vi "2636 EPSC LTP LTD Cycles.vi"() -> ()   [LabVIEW 2023]
uses:
  <instrlib>/Keithley 2600 Series/Public/Channel.ctl
  <instrlib>/Keithley 2600 Series/Keithley 2600 Series.lvlib
  <userlib>/_OpenG.lib/time/time.llb/openg_time.lvlib
panel:
  in  "Cycle Number":u32=50
  in  "LTD Pulse Level (V)":dbl=-10.0
  in  "error in (no error)":errorcluster
  in  "Log Time After Pulses (s)":dbl=0.5 format="%#_13g"
  in  "Log Time Before Pulses (s)":dbl=0.5 format="%#_13g"
  in  "Auto Enable Output":bool=TRUE
  in  "Reset":bool=TRUE
  in  "Error Query":bool
  out "Pulsed IV Filename Out":path caption="Filename Out"
  in  "Pulsed IV Filename":path=path "C:/Data/pulse_I_V.lvm" caption="Filename"
  out "Pulse IV":cluster{"X":dbl[], "Y":dbl[]}[](graph)
  out "I_ds Log Filename Out":path caption="Filename Out"
  in  "I_ds Log Filename":path=path "C:/Data/I_ds_vs_time.lvm" caption="Filename"
  out "Data":dbl[](array[numeric])
  out "Result Chart":dynamicdata(graph)
  out "error out":errorcluster
  out "Complete?":bool
  out "Overflow?":bool
  in  "Stop":bool
  in  "Pulse Duration (s)":dbl=0.01
  in  "Post-Pulse Duration (s)":dbl=0.05
  in  "Pre-Pulse Duration (s)":dbl=0.05
  in  "Buffer size":u32=1024
  in  "LT Pulse Number":u32=50
  in  "Drain Source Channel":T1=enum."Channel B"
  in  "V_ds(V)":dbl=0.01
  in  "I_ds NPLC":dbl=0.1
  in  "I_ds Range (A)":dbl=1e-06
  in  "I pulse Range (A)":dbl=1e-06
  in  "I pulse NPLC":dbl=0.1
  in  "LTP Pulse Level (V)":dbl=10.0
  in  "Pulse Channel":T1
  in  "2636 Address":refnum<visa-resource-name>="GPIB0::26::INSTR"
  # "Synaptic EPSC LTP-LTD Cycle Test (Three-terminal Devices)"
  # "by JHC (20250322)"
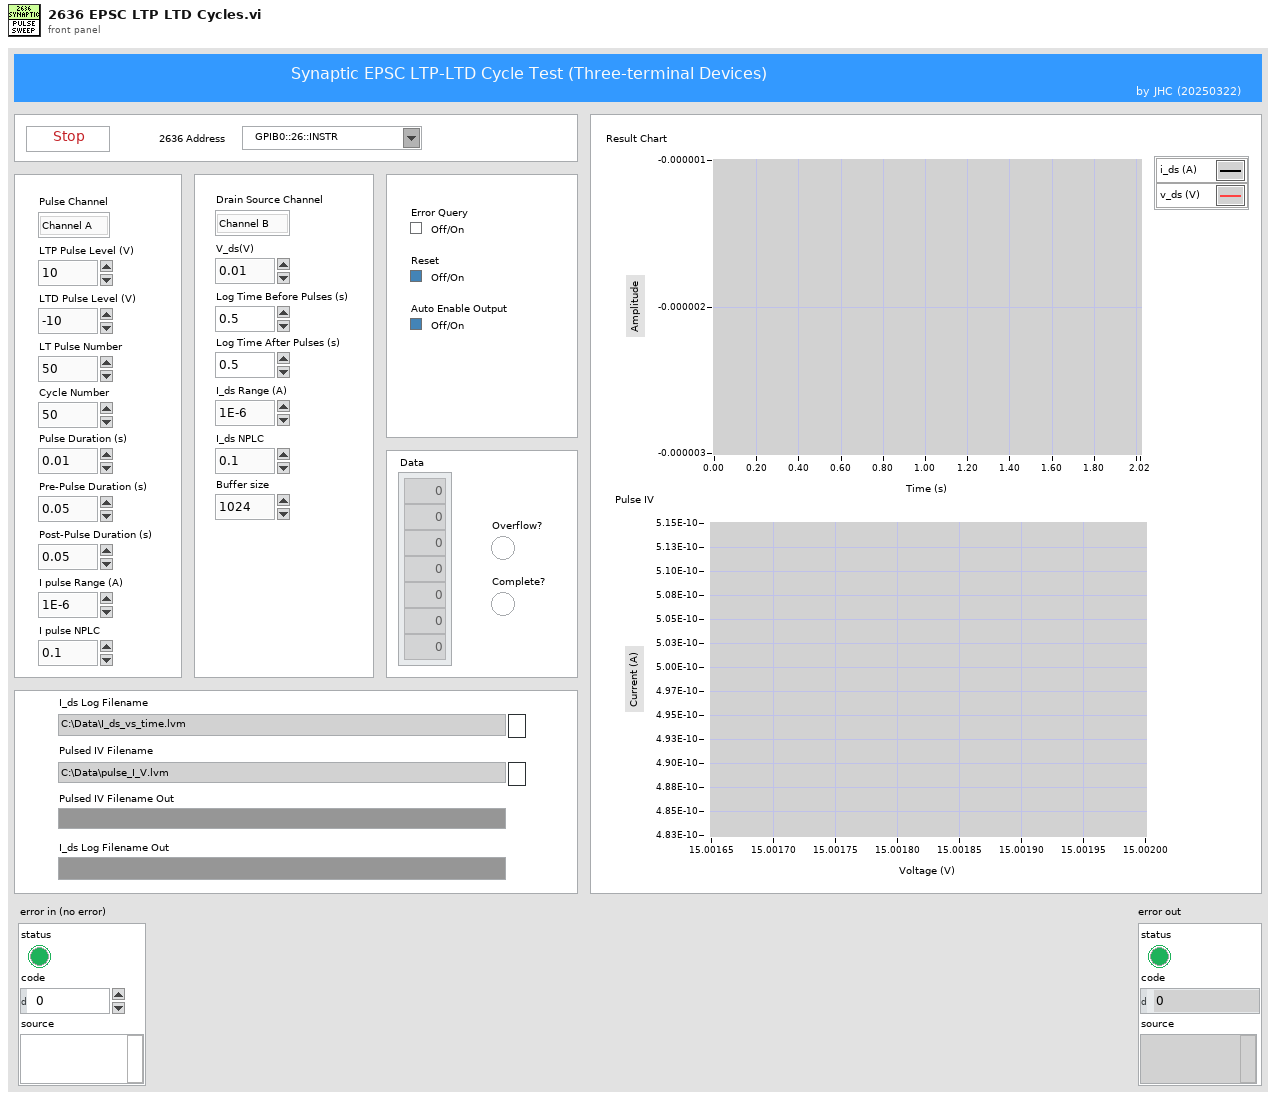
[diagram p1: front panel]
types:
  T1 = typedef "Keithley 2600 Series.lvlib/Channel.ctl" = enum32{"Channel A", "Channel B"}
  T2 = enum16{"None/Disconnect", "Digital I/O Trigger", "TSP-Link Trigger", "LAN Trigger", "Blender", "Timer Expired", "Front Panel Trigger", "Software Trigger", "SMU Sweeping", "SMU Armed", "SMU Source Complete", "SMU Measure Complete", "SMU Pulse Complete", "SMU Sweep Complete", "SMU Idle"}
  T3 = enum16{"Current", "Voltage", "IV", "Resistance", "Power"}
  T4 = enum32{"ASCII", "Real 32", "Real 64", "Single Precision Real", "Double Precision Real"}
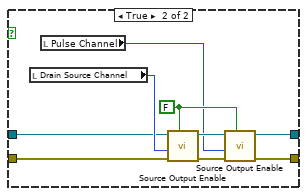
[diagram p2: hidden frame]
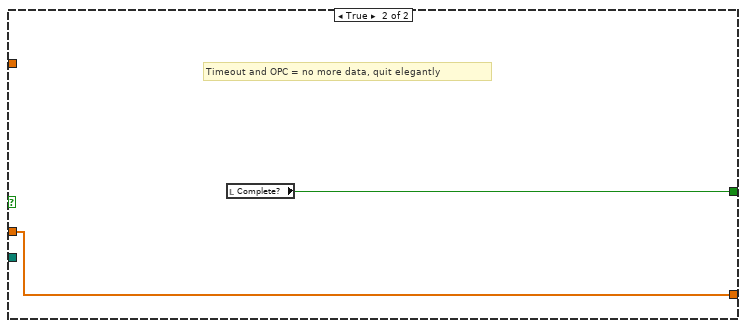
[diagram p5: hidden frame]
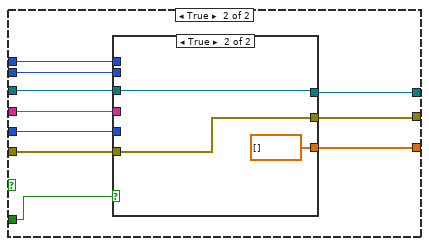
[diagram p8: hidden frame]
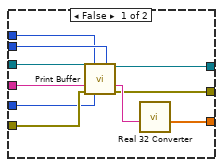
[diagram p9: hidden frame]
diagram:
  w19 = sgl[] [] ("Data Array Out")
  w22 = u16 1 items=["Channel A", "Channel B"] ("Channel (Channel A)")
  w23 = u16 0 items=["Channel A", "Channel B"] ("Channel (Channel A)")
  w39 = u16 0 items=["Current", "Voltage", "Resistance", "Power"] ("Function (Current)")
  w47 = u16 2 items=["Channel A", "Channel B", "Channels A & B", "User"] ("Screen (Channels A & B)")
  # "Wait 1s"
  # "Start Pulse SMU"
  # "Start DS SMU"
  n1 = call <instrlib>:"Initialize.vi"("Reset (True)"="Reset", "error in (no error)"="error in (no error)", "Error Query (False)"="Error Query", "ID Query (True)"=TRUE, "VISA resource name"="2636 Address") -> ("error out"=w2:errorcluster, "VISA resource name out"=w5:refnum<visa-resource-name>)  [unwired: 5 in]
  n2 = call <instrlib>:"Error Queue Clear.vi"("error in (no error)"=w2, "VISA resource name"=w5) -> ("error out"=w3:errorcluster, "VISA resource name out"=w4:refnum<visa-resource-name>)  [unwired: 6 in, 2 out]
  n3 = call <instrlib>:"Abort SMU Op.vi"("error in"=w3, "Channel (Channel A)"=w23, "VISA resource name"=w4) -> ("error out"=w24:errorcluster, "VISA resource name out"=w25:refnum<visa-resource-name>)  [unwired: 5 in, 2 out]
  n4 = call <instrlib>:"Abort SMU Op.vi"("error in"=w24, "Channel (Channel A)"=w22, "VISA resource name"=w25) -> ("error out"=w20:errorcluster, "VISA resource name out"=w21:refnum<visa-resource-name>)  [unwired: 5 in, 2 out]
  n5 = call <instrlib>:"Reset SMU.vi"("SMU B (No)"="Reset", "SMU A (No)"="Reset", "error in (no error)"=w20, "VISA resource name"=w21) -> ("error out"=w86:errorcluster, "VISA resource name out"=w87:refnum<visa-resource-name>)  [unwired: 4 in, 2 out]
  n6 = flat-sequence {
    tunnel: w87 -> [w120]
    tunnel: w86 -> [w119]
    tunnel: [w101] -> w85
    tunnel: [w100] -> w84
    tunnel: w85 -> [w143]
    tunnel: w84 -> [w144]
    tunnel: [w142] -> w83
    tunnel: [w141] -> w82
    tunnel: w83 -> [w185]
    tunnel: w82 -> [w183]
    tunnel: [w164] -> w81
    tunnel: [w163] -> w80
    tunnel: w81 -> [w273]
    tunnel: w80 -> [w272]
    tunnel: [w240] -> w79
    tunnel: [w239] -> w78
    tunnel: [w227] -> w77
    tunnel: w79 -> [w307]
    tunnel: w78 -> [w308]
    tunnel: w77 -> [w330]
    tunnel: [w311] -> w76
    tunnel: [w310] -> w75
    tunnel: w76 -> [w338]
    tunnel: w75 -> [w337]
    tunnel: [w334] -> w44
    tunnel: [w333] -> w43
    frame #0 {
      w108 = enum32{"Current", "Voltage"}."Current" ("Function (Current)")
      w109 = FALSE ("Autorange (On)")
      w89 = enum32{"Current", "Voltage"}."Voltage" ("Function (Current)")
      # "Init Pulse Gate Channel"
      n7 = call <instrlib>:"Source Function.vi"("Function (Current)"=w89, "error in (no error)"=w119, "Channel (Channel A)"="Pulse Channel", "VISA resource name"=w120) -> ("error out"=w121:errorcluster, "VISA resource name out"=w122:refnum<visa-resource-name>)  [unwired: 4 in, 2 out]
      n8 = call <instrlib>:"Source Level.vi"("Level (0.000)"=0.0, "Function (Current)"=w89, "error in (no error)"=w121, "Channel (Channel A)"="Pulse Channel", "VISA resource name"=w122) -> ("error out"=w117:errorcluster, "VISA resource name out"=w118:refnum<visa-resource-name>)  [unwired: 3 in, 2 out]
      n9 = call <instrlib>:"Source Autorange.vi"("Autorange (On)"=w109, "Function (Current)"=w89, "error in (no error)"=w117, "Channel (Channel A)"="Pulse Channel", "VISA resource name"=w118) -> ("error out"=w115:errorcluster, "VISA resource name out"=w116:refnum<visa-resource-name>)  [unwired: 3 in, 2 out]
      n10 = local read "LTP Pulse Level (V)"() -> (w88:dbl)
      n11 = call <instrlib>:"Source Autorange.vi"("Autorange (On)"=w109, "Function (Current)"=w108, "error in (no error)"=w115, "Channel (Channel A)"="Pulse Channel", "VISA resource name"=w116) -> ("error out"=w96:errorcluster, "VISA resource name out"=w98:refnum<visa-resource-name>)  [unwired: 3 in, 2 out]
      n12 = call <instrlib>:"Source Range.vi"("Range (1.000)"=w88, "Function (Current)"=w89, "error in (no error)"=w96, "Channel (Channel A)"="Pulse Channel", "VISA resource name"=w98) -> ("error out"=w95:errorcluster, "VISA resource name out"=w97:refnum<visa-resource-name>)  [unwired: 3 in, 2 out]
      n13 = call <instrlib>:"Measure NPLC.vi"("NPLC (1.000)"="I pulse NPLC", "error in (no error)"=w95, "Channel (Channel A)"="Pulse Channel", "VISA resource name"=w97) -> ("error out"=w113:errorcluster, "VISA resource name out"=w110:refnum<visa-resource-name>)  [unwired: 4 in, 2 out]
      n14 = call <instrlib>:"Measure Autorange.vi"("Autorange (On)"=w109, "Function (Current)"=w89, "error in (no error)"=w113, "Channel (Channel A)"="Pulse Channel", "VISA resource name"=w110) -> ("error out"=w112:errorcluster, "VISA resource name out"=w111:refnum<visa-resource-name>)  [unwired: 3 in, 2 out]
      n15 = call <instrlib>:"Measure Autorange.vi"("Autorange (On)"=w109, "Function (Current)"=w108, "error in (no error)"=w112, "Channel (Channel A)"="Pulse Channel", "VISA resource name"=w111) -> ("error out"=w94:errorcluster, "VISA resource name out"=w93:refnum<visa-resource-name>)  [unwired: 3 in, 2 out]
      n16 = call <instrlib>:"Measure Range.vi"("Range (1.000)"=w88, "Function (Current)"=w89, "error in (no error)"=w94, "Channel (Channel A)"="Pulse Channel", "VISA resource name"=w93) -> ("error out"=w91:errorcluster, "VISA resource name out"=w92:refnum<visa-resource-name>)  [unwired: 3 in, 2 out]
      n17 = call <instrlib>:"Measure Range.vi"("Range (1.000)"="I pulse Range (A)", "Function (Current)"=w108, "error in (no error)"=w91, "Channel (Channel A)"="Pulse Channel", "VISA resource name"=w92) -> ("error out"=w106:errorcluster, "VISA resource name out"=w105:refnum<visa-resource-name>)  [unwired: 3 in, 2 out]
      n18 = call <instrlib>:"Measure Sense Mode.vi"("error in (no error)"=w106, "Channel (Channel A)"="Pulse Channel", "VISA resource name"=w105) -> ("error out"=w103:errorcluster, "VISA resource name out"=w104:refnum<visa-resource-name>)  [unwired: 2 in, 5 out]
      n19 = call <instrlib>:"Measure Autozero.vi"("Autozero (Auto)"=enum32{"Off", "Once", "Auto"}."Once", "error in (no error)"=w103, "Channel (Channel A)"="Pulse Channel", "VISA resource name"=w104) -> ("error out"=w100:errorcluster, "VISA resource name out"=w101:refnum<visa-resource-name>)  [unwired: 1 in, 5 out]
    }
    frame #1 {
      w126 = 0.0 ("Interval (0.000)")
      w146 = enum32{"Current", "Voltage"}."Current" ("Function (Current)")
      w145 = FALSE ("Autorange (On)")
      w132 = enum32{"Current", "Voltage"}."Voltage" ("Function (Current)")
      # "Init Drain Source Channel"
      n20 = call <instrlib>:"Source Function.vi"("Function (Current)"=w132, "error in (no error)"=w144, "Channel (Channel A)"="Drain Source Channel", "VISA resource name"=w143) -> ("error out"=w160:errorcluster, "VISA resource name out"=w161:refnum<visa-resource-name>)  [unwired: 4 in, 2 out]
      n21 = call <instrlib>:"Source Level.vi"("Level (0.000)"="V_ds(V)", "Function (Current)"=w132, "error in (no error)"=w160, "Channel (Channel A)"="Drain Source Channel", "VISA resource name"=w161) -> ("error out"=w158:errorcluster, "VISA resource name out"=w159:refnum<visa-resource-name>)  [unwired: 3 in, 2 out]
      n22 = call <instrlib>:"Source Autorange.vi"("Autorange (On)"=w145, "Function (Current)"=w132, "error in (no error)"=w158, "Channel (Channel A)"="Drain Source Channel", "VISA resource name"=w159) -> ("error out"=w156:errorcluster, "VISA resource name out"=w157:refnum<visa-resource-name>)  [unwired: 3 in, 2 out]
      n23 = call <instrlib>:"Source Autorange.vi"("Autorange (On)"=w145, "Function (Current)"=w146, "error in (no error)"=w156, "Channel (Channel A)"="Drain Source Channel", "VISA resource name"=w157) -> ("error out"=w140:errorcluster, "VISA resource name out"=w137:refnum<visa-resource-name>)  [unwired: 3 in, 2 out]
      n24 = call <instrlib>:"Source Range.vi"("Range (1.000)"="V_ds(V)", "Function (Current)"=w132, "error in (no error)"=w140, "Channel (Channel A)"="Drain Source Channel", "VISA resource name"=w137) -> ("error out"=w139:errorcluster, "VISA resource name out"=w138:refnum<visa-resource-name>)  [unwired: 3 in, 2 out]
      n25 = call <instrlib>:"Measure NPLC.vi"("NPLC (1.000)"="I_ds NPLC", "error in (no error)"=w139, "Channel (Channel A)"="Drain Source Channel", "VISA resource name"=w138) -> ("error out"=w127:errorcluster, "VISA resource name out"=w128:refnum<visa-resource-name>)  [unwired: 4 in, 2 out]
      n26 = call <instrlib>:"Measure Interval.vi"("Interval (0.000)"=w126, "error in (no error)"=w127, "Channel (Channel A)"="Drain Source Channel", "VISA resource name"=w128) -> ("error out"=w130:errorcluster, "VISA resource name out"=w129:refnum<visa-resource-name>)  [unwired: 4 in, 2 out]
      n27 = call <instrlib>:"Measure Delay.vi"("Delay (0)"=w126, "error in (no error)"=w130, "Channel (Channel A)"="Drain Source Channel", "VISA resource name"=w129) -> ("error out"=w124:errorcluster, "VISA resource name out"=w125:refnum<visa-resource-name>)  [unwired: 4 in, 2 out]
      n28 = call <instrlib>:"Measure Autorange.vi"("Autorange (On)"=w145, "Function (Current)"=w132, "error in (no error)"=w124, "Channel (Channel A)"="Drain Source Channel", "VISA resource name"=w125) -> ("error out"=w154:errorcluster, "VISA resource name out"=w153:refnum<visa-resource-name>)  [unwired: 3 in, 2 out]
      n29 = call <instrlib>:"Measure Autorange.vi"("Autorange (On)"=w145, "Function (Current)"=w146, "error in (no error)"=w154, "Channel (Channel A)"="Drain Source Channel", "VISA resource name"=w153) -> ("error out"=w133:errorcluster, "VISA resource name out"=w134:refnum<visa-resource-name>)  [unwired: 3 in, 2 out]
      n30 = call <instrlib>:"Measure Range.vi"("Range (1.000)"="V_ds(V)", "Function (Current)"=w132, "error in (no error)"=w133, "Channel (Channel A)"="Drain Source Channel", "VISA resource name"=w134) -> ("error out"=w136:errorcluster, "VISA resource name out"=w135:refnum<visa-resource-name>)  [unwired: 3 in, 2 out]
      n31 = call <instrlib>:"Measure Range.vi"("Range (1.000)"="I_ds Range (A)", "Function (Current)"=w146, "error in (no error)"=w136, "VISA resource name"=w135) -> ("error out"=w151:errorcluster, "VISA resource name out"=w150:refnum<visa-resource-name>)  [unwired: 4 in, 2 out]
      n32 = call <instrlib>:"Measure Sense Mode.vi"("error in (no error)"=w151, "Channel (Channel A)"="Drain Source Channel", "VISA resource name"=w150) -> ("error out"=w148:errorcluster, "VISA resource name out"=w149:refnum<visa-resource-name>)  [unwired: 2 in, 5 out]
      n33 = call <instrlib>:"Measure Autozero.vi"("Autozero (Auto)"=enum32{"Off", "Once", "Auto"}."Once", "error in (no error)"=w148, "Channel (Channel A)"="Drain Source Channel", "VISA resource name"=w149) -> ("error out"=w142:errorcluster, "VISA resource name out"=w141:refnum<visa-resource-name>)  [unwired: 1 in, 5 out]
    }
    frame #2 {
      w177 = TRUE ("Append Mode (Off)")
      w176 = "v_ds" ("Buffer Name (buf)")
      w178 = TRUE ("Append Mode (Off)")
      w180 = "i_ds" ("Buffer Name (buf)")
      w189 = FALSE ("Collect Timestamps (Off)")
      w188 = "pulse_iv_table.v" ("Buffer Name (buf)")
      w187 = TRUE ("Append Mode (Off)")
      w186 = "pulse_iv_table.i" ("Buffer Name (buf)")
      # "set up circular buffer"
      # "A large size"
      # "Init Buffer"
      n34 = local read "Pulse Channel"() -> (w204:T1)
      n35 = local read "LT Pulse Number"() -> (w162:u32)
      n36 = VISA Write(VISA resource name=w183, write buffer="pulse_iv_table = {}\nds_iv_table = {}", error in (no error)=w185) -> (VISA resource name out=w190:refnum<visa-resource-name>, error out=w191:errorcluster)  [unwired: 1 out]
      n37 = call <instrlib>:"Error Query.vi"("error in (no error)"=w191, "VISA resource name"=w190) -> ("error out"=w203:errorcluster, "VISA resource name out"=w202:refnum<visa-resource-name>)  [unwired: 8 out]
      n38 = call <instrlib>:"Buffer Make Buffer.vi"("Capacity (1)"=w162, "Channel (Channel A)"=w204, "error in (no error)"=w203, "Buffer Name (buf)"=w186, "VISA resource name"=w202) -> ("error out"=w192:errorcluster, "VISA resource name out"=w193:refnum<visa-resource-name>)  [unwired: 1 in, 4 out]
      n39 = call <instrlib>:"Buffer Clear.vi"("error in (no error)"=w192, "Buffer Name"=w186, "VISA resource name"=w193) -> ("error out"=w195:errorcluster, "VISA resource name out"=w194:refnum<visa-resource-name>)  [unwired: 7 out]
      n40 = call <instrlib>:"Buffer Configure.vi"("Collect Timestamps (Off)"=w189, "error in (no error)"=w195, "Buffer Name"=w186, "Append Mode (Off)"=w187, "VISA resource name"=w194) -> ("error out"=w197:errorcluster, "VISA resource name out"=w196:refnum<visa-resource-name>)  [unwired: 2 in, 3 out]
      n41 = call <instrlib>:"Buffer Make Buffer.vi"("Capacity (1)"=w162, "Channel (Channel A)"=w204, "error in (no error)"=w197, "Buffer Name (buf)"=w188, "VISA resource name"=w196) -> ("error out"=w199:errorcluster, "VISA resource name out"=w198:refnum<visa-resource-name>)  [unwired: 1 in, 4 out]
      n42 = call <instrlib>:"Buffer Clear.vi"("error in (no error)"=w199, "Buffer Name"=w188, "VISA resource name"=w198) -> ("error out"=w201:errorcluster, "VISA resource name out"=w200:refnum<visa-resource-name>)  [unwired: 7 out]
      n43 = call <instrlib>:"Buffer Configure.vi"("Collect Source Values (Off)"=w189, "error in (no error)"=w201, "Buffer Name"=w188, "Append Mode (Off)"=w187, "VISA resource name"=w200) -> ("error out"=w210:errorcluster, "VISA resource name out"=w209:refnum<visa-resource-name>)  [unwired: 2 in, 3 out]
      n44 = local read "Drain Source Channel"() -> (w168:T1)
      n45 = call <instrlib>:"Buffer Make Buffer.vi"("Capacity (1)"="Buffer size", "Channel (Channel A)"=w168, "error in (no error)"=w210, "Buffer Name (buf)"=w180, "VISA resource name"=w209) -> ("error out"=w206:errorcluster, "VISA resource name out"=w205:refnum<visa-resource-name>)  [unwired: 1 in, 4 out]
      n46 = call <instrlib>:"Buffer Clear.vi"("error in (no error)"=w206, "Buffer Name"=w180, "VISA resource name"=w205) -> ("error out"=w208:errorcluster, "VISA resource name out"=w207:refnum<visa-resource-name>)  [unwired: 7 out]
      n47 = call <instrlib>:"Buffer Configure.vi"("Collect Timestamps (Off)"=w178, "error in (no error)"=w208, "Buffer Name"=w180, "Append Mode (Off)"=w178, "VISA resource name"=w207) -> ("error out"=w182:errorcluster, "VISA resource name out"=w181:refnum<visa-resource-name>)  [unwired: 2 in, 3 out]
      n48 = call <instrlib>:"Advanced Buffer Configuration.vi"("VISA resource name"=w181, "Enable Buffer Cache Mode (Disable)"=w178, "Buffer Name"=w180, "Buffer Fill Mode (Fill_Once)"=enum16{"FILL_ONCE", "FILL_WINDOW"}."FILL_WINDOW", "error in (no error)"=w182) -> ("VISA resource name out"=w166:refnum<visa-resource-name>, "error out"=w165:errorcluster)  [unwired: 9 in]
      n49 = call <instrlib>:"Buffer Make Buffer.vi"("Capacity (1)"="Buffer size", "Channel (Channel A)"=w168, "error in (no error)"=w165, "Buffer Name (buf)"=w176, "VISA resource name"=w166) -> ("error out"=w172:errorcluster, "VISA resource name out"=w173:refnum<visa-resource-name>)  [unwired: 1 in, 4 out]
      n50 = call <instrlib>:"Buffer Clear.vi"("error in (no error)"=w172, "Buffer Name"=w176, "VISA resource name"=w173) -> ("error out"=w170:errorcluster, "VISA resource name out"=w171:refnum<visa-resource-name>)  [unwired: 7 out]
      n51 = call <instrlib>:"Buffer Configure.vi"("Collect Timestamps (Off)"=w177, "error in (no error)"=w170, "Buffer Name"=w176, "Append Mode (Off)"=w177, "VISA resource name"=w171) -> ("error out"=w174:errorcluster, "VISA resource name out"=w175:refnum<visa-resource-name>)  [unwired: 2 in, 3 out]
      n52 = call <instrlib>:"Advanced Buffer Configuration.vi"("VISA resource name"=w175, "Enable Buffer Cache Mode (Disable)"=w177, "Buffer Name"=w176, "Buffer Fill Mode (Fill_Once)"=enum16{"FILL_ONCE", "FILL_WINDOW"}."FILL_WINDOW", "error in (no error)"=w174) -> ("VISA resource name out"=w163:refnum<visa-resource-name>, "error out"=w164:errorcluster)  [unwired: 9 in]
    }
    frame #3 {
      w231 = u32 4 ("Timer Number (1)")
      w243 = u32 1 ("Timer Number (1)")
      w255 = u32 3 ("Timer Number (1)")
      w278 = u32 2 ("Timer Number (1)")
      # "SMU Armed when timer4 expires"
      # "Trigger timer4 when the SMU Sweeping, only once"
      # "Trigger timer1 when the SMU Armed, repeat N times"
      # "Trigger end pulse after timer3 expired"
      # "Configure measure action (default is 0) to start after source immediately"
      # "set source pulse level and end pusle idle"
      # "Trigger timer3 when the SMU source pulse level"
      # "Create a fixed level voltage sweep"
      # "Configure source action to start after timer2 expired"
      # "Trigger timer2 when timer1 expired or first run."
      # "Init Trigger Model (Pulse Channel)"
      n53 = for {
        N: "LT Pulse Number" -> [_]
        tunnel: "LTP Pulse Level (V)" -> [w287]
        tunnel: "LTD Pulse Level (V)" -> [w286]
        tunnel: [w287] -> w217 mode=indexing
        tunnel: [w286] -> w216 mode=indexing
      }
      n54 = Build Array(w217, w216) -> (w215:dbl[][])
      n55 = Array To Spreadsheet String(delimiter (Tab)=",", array=w215, 3:"%f" ("format string")) -> (spreadsheet string=w218:string)
      n56 = local read "Pulse Channel"() -> (w227:T1)
      n57 = Pick Line(multi-line string="smua\nsmub", line index=w227) -> (output string=w238:string)  [unwired: 1 in]
      n58 = Format Into String(format string="%s.trigger.source.listv({%s})\\n", w238, w218) -> (resulting string=w276:string)  [unwired: 2 in, 1 out]
      n59 = call <instrlib>:"Format Event ID.vi"("Channel (Channel A)"=w227, "Event Type (None)"=T2."SMU Sweeping") -> ("Event ID"=w235:string)  [unwired: 8 in, 1 out]
      n60 = Format Into String(format string="%s.trigger.source.action = %s.ENABLE\n%s.trigger.endpulse.action = %s.SOURCE_IDLE", initial string=w276, w238, w238, w238, w238) -> (resulting string=w271:string)  [unwired: 1 in, 1 out]
      n61 = VISA Write(VISA resource name=w272, write buffer=w271, error in (no error)=w273) -> (VISA resource name out=w237:refnum<visa-resource-name>, error out=w236:errorcluster)  [unwired: 1 out]
      n62 = call <instrlib>:"Config Timer.vi"("VISA resource name"=w237, "Delay (1e-3)"="Log Time Before Pulses (s)", "Timer Number (1)"=w231, "error in"=w236, "Input Event"=w235) -> ("VISA resource name out"=w233:refnum<visa-resource-name>, "error out"=w229:errorcluster)  [unwired: 7 in, 2 out]
      n63 = call <instrlib>:"Format Event ID.vi"("Event Module # (1)"=w231, "Event Type (None)"=T2."Timer Expired") -> ("Event ID"=w230:string)  [unwired: 8 in, 1 out]
      n64 = call <instrlib>:"Config Arm Event.vi"("Arm Input Event"=w230, "error in"=w229, "Channel (Channel A)"=w227, "VISA resource name"=w233) -> ("error out"=w225:errorcluster, "VISA resource name out"=w224:refnum<visa-resource-name>)  [unwired: 4 in, 2 out]
      n65 = call <instrlib>:"Format Event ID.vi"("Channel (Channel A)"=w227, "Event Type (None)"=T2."SMU Armed") -> ("Event ID"=w226:string)  [unwired: 8 in, 1 out]
      n66 = local read "LT Pulse Number"() -> (w248:u32)
      n67 = local read "Pre-Pulse Duration (s)"() -> (w252:dbl)
      n68 = local read "Pulse Duration (s)"() -> (w253:dbl)
      n69 = Decrement(x=w248) -> (x-1=w244:u32)
      n70 = Compound Arithmetic op=ADD(w253, w252, "Post-Pulse Duration (s)") -> (w250:dbl)
      n71 = call <instrlib>:"Config Timer.vi"("VISA resource name"=w224, "Count (1)"=w244, "Delay (1e-3)"=w250, "Timer Number (1)"=w243, "Passthrough (Off)"=TRUE, "error in"=w225, "Input Event"=w226) -> ("VISA resource name out"=w245:refnum<visa-resource-name>, "error out"=w246:errorcluster)  [unwired: 5 in, 2 out]
      n72 = call <instrlib>:"Format Event ID.vi"("Event Module # (1)"=w243, "Event Type (None)"=T2."Timer Expired") -> ("Event ID"=w282:string)  [unwired: 8 in, 1 out]
      n73 = call <instrlib>:"Config Timer.vi"("VISA resource name"=w245, "Delay (1e-3)"="Pre-Pulse Duration (s)", "Timer Number (1)"=w278, "error in"=w246, "Input Event"=w282) -> ("VISA resource name out"=w281:refnum<visa-resource-name>, "error out"=w280:errorcluster)  [unwired: 7 in, 2 out]
      n74 = call <instrlib>:"Format Event ID.vi"("Event Module # (1)"=w278, "Event Type (None)"=T2."Timer Expired") -> ("Event ID"=w277:string)  [unwired: 8 in, 1 out]
      n75 = call <instrlib>:"Config Source Event.vi"("Input Event"=w277, "error in"=w280, "Channel (Channel A)"=w227, "VISA resource name"=w281) -> ("error out"=w266:errorcluster, "VISA resource name out"=w267:refnum<visa-resource-name>)  [unwired: 4 in, 2 out]
      n76 = call <instrlib>:"Format Event ID.vi"("Channel (Channel A)"=w227, "Event Type (None)"=T2."SMU Source Complete") -> ("Event ID"=w269:string)  [unwired: 8 in, 1 out]
      n77 = call <instrlib>:"Config Timer.vi"("VISA resource name"=w267, "Delay (1e-3)"="Pulse Duration (s)", "Timer Number (1)"=w255, "error in"=w266, "Input Event"=w269) -> ("VISA resource name out"=w265:refnum<visa-resource-name>, "error out"=w264:errorcluster)  [unwired: 7 in, 2 out]
      n78 = local read "LT Pulse Number"() -> (w213:u32)
      n79 = call <instrlib>:"Config Measure Event.vi"("VISA resource name"=w265, "Configure Measurement (Disable)"=enum8{"DISABLE", "ENABLE", "ASYNC"}."ENABLE", "Buffer 1"="pulse_iv_table.i" ("Buffer Name (buf)"), "Buffer 2"="pulse_iv_table.v" ("Buffer Name (buf)"), "Channel (Channel A)"=w227, "Function (Current)"=T3."IV", "error in"=w264, "Measure Input Event"="0") -> ("VISA resource name out"=w258:refnum<visa-resource-name>, "error out"=w257:errorcluster)  [unwired: 4 in, 2 out]
      n80 = call <instrlib>:"Format Event ID.vi"("Event Module # (1)"=w255, "Event Type (None)"=T2."Timer Expired") -> ("Event ID"=w254:string)  [unwired: 8 in, 1 out]
      n81 = call <instrlib>:"Config End Pulse Event.vi"("Input Event"=w254, "error in"=w257, "Channel (Channel A)"=w227, "VISA resource name"=w258) -> ("error out"=w242:errorcluster, "VISA resource name out"=w241:refnum<visa-resource-name>)  [unwired: 4 in, 2 out]
      n82 = Multiply(x=u32 2, y=w213) -> (x*y=w211:u32)
      n83 = call <instrlib>:"Config Layer Count.vi"("Trigger Count (1)"=w211, "Arm Count (1)"="Cycle Number", "error in"=w242, "Channel (Channel A)"=w227, "VISA resource name"=w241) -> ("error out"=w239:errorcluster, "VISA resource name out"=w240:refnum<visa-resource-name>)  [unwired: 3 in, 2 out]
    }
    frame #4 {
      w292 = u32 5 ("Timer Number (1)")
      w320 = u32 1 ("Blender Number (1)")
      # "BUG from Driver: if Async, measure.Y is not set"
      # "No trigger, start\nasync measure after SMU Armed, as fast as possible"
      # "Trigger timer5 when Pulse SMU Idle\nto keep measure for a while"
      # "Blend two events from Pulse SMU to trigger DS SMU Source action\nDS SMU Source start when Pulse SMU start sweeping\nWhen Pulse SMU become idle, DS SMU source again and stop"
      # "set source level, and hold"
      # "Create a fixed level voltage sweep"
      # "Init Trigger Model (Drain Source Channel)"
      n84 = local read "Drain Source Channel"() -> (w313:T1)
      n85 = local read "V_ds(V)"() -> (w324:dbl)
      n86 = Pick Line(multi-line string="smua\nsmub", line index=w313) -> (output string=w300:string)  [unwired: 1 in]
      n87 = Format Into String(format string="%s.trigger.source.listv({%f})\\n", w300, w324) -> (resulting string=w327:string)  [unwired: 2 in, 1 out]
      n88 = Format Into String(format string="%s.trigger.source.action = %s.ENABLE\n%s.trigger.endpulse.action = %s.SOURCE_HOLD", initial string=w327, w300, w300, w300, w300) -> (resulting string=w306:string)  [unwired: 1 in, 1 out]
      n89 = VISA Write(VISA resource name=w307, write buffer=w306, error in (no error)=w308) -> (VISA resource name out=w296:refnum<visa-resource-name>, error out=w297:errorcluster)  [unwired: 1 out]
      n90 = call <instrlib>:"Format Event ID.vi"("Channel (Channel A)"=w330, "Event Type (None)"=T2."SMU Sweeping") -> ("Event ID"=w291:string)  [unwired: 8 in, 1 out]
      n91 = call <instrlib>:"Format Event ID.vi"("Channel (Channel A)"=w330, "Event Type (None)"=T2."SMU Idle") -> ("Event ID"=w294:string)  [unwired: 8 in, 1 out]
      n92 = call <instrlib>:"Config Timer.vi"("VISA resource name"=w296, "Delay (1e-3)"="Log Time After Pulses (s)", "Timer Number (1)"=w292, "error in"=w297, "Input Event"=w294) -> ("VISA resource name out"=w288:refnum<visa-resource-name>, "error out"=w289:errorcluster)  [unwired: 7 in, 2 out]
      n93 = call <instrlib>:"Format Event ID.vi"("Event Module # (1)"=w292, "Event Type (None)"=T2."Timer Expired") -> ("Event ID"=w290:string)  [unwired: 8 in, 1 out]
      n94 = call <instrlib>:"Config Event Blender.vi"("VISA resource name"=w288, "Input Event 1"=w290, "Input Event 2"=w291, "Blender Number (1)"=w320, "Blend Type (OR)"=enum16{"OR", "AND"}."OR", "error in"=w289) -> ("VISA resource name out"=w322:refnum<visa-resource-name>, "error out"=w323:errorcluster)  [unwired: 6 in, 2 out]
      n95 = call <instrlib>:"Format Event ID.vi"("Event Module # (1)"=w320, "Event Type (None)"=T2."Blender") -> ("Event ID"=w319:string)  [unwired: 8 in, 1 out]
      n96 = call <instrlib>:"Config Source Event.vi"("Input Event"=w319, "error in"=w323, "Channel (Channel A)"=w313, "VISA resource name"=w322) -> ("error out"=w316:errorcluster, "VISA resource name out"=w317:refnum<visa-resource-name>)  [unwired: 4 in, 2 out]
      n97 = call <instrlib>:"Config Measure Event.vi"("VISA resource name"=w317, "Configure Measurement (Disable)"=enum8{"DISABLE", "ENABLE", "ASYNC"}."ENABLE", "Buffer 1"="i_ds" ("Buffer Name (buf)"), "Buffer 2"="v_ds" ("Buffer Name (buf)"), "Channel (Channel A)"=w313, "Function (Current)"=T3."IV", "error in"=w316) -> ("VISA resource name out"=w302:refnum<visa-resource-name>, "error out"=w303:errorcluster)  [unwired: 5 in, 2 out]
      n98 = Format Into String(format string="%s.trigger.measure.action = %s.ASYNC", w300, w300) -> (resulting string=w299:string)  [unwired: 2 in, 1 out]
      n99 = VISA Write(VISA resource name=w302, write buffer=w299, error in (no error)=w303) -> (VISA resource name out=w305:refnum<visa-resource-name>, error out=w304:errorcluster)  [unwired: 1 out]
      n100 = call <instrlib>:"Config Layer Count.vi"("Trigger Count (1)"=u32 2 ("Arm Count (1)"), "Arm Count (1)"=u32 1, "error in"=w304, "Channel (Channel A)"=w313, "VISA resource name"=w305) -> ("error out"=w310:errorcluster, "VISA resource name out"=w311:refnum<visa-resource-name>)  [unwired: 3 in, 2 out]
    }
    frame #5 {
      # "Other init jobs"
      n101 = call <instrlib>:"Data Output Format.vi"("ASCII Precision (6)"=6, "error in (no error)"=w337, "Data Format (ASCII)"=T4."Real 32", "VISA resource name"=w338) -> ("error out"=w333:errorcluster, "VISA resource name out"=w334:refnum<visa-resource-name>)  [unwired: 4 in, 2 out]
    }
  }
  n102 = local read "Pulse Channel"() -> (w41:T1)
  n103 = local read "Drain Source Channel"() -> (w40:T1)
  n104 = call <instrlib>:"Display Screen.vi"("Screen (Channels A & B)"=w47, "error in (no error)"=w43, "VISA resource name"=w44) -> ("error out"=w50:errorcluster, "Node Out"=w49:string, "VISA resource name out"=w48:refnum<visa-resource-name>)  [unwired: 5 in, 1 out]
  n105 = call <instrlib>:"Display Measure Function.vi"("Function (Current)"=w39, "error in (no error)"=w50, "Channel (Channel A)"=w41, "Node In"=w49, "VISA resource name"=w48) -> ("error out"=w46:errorcluster, "VISA resource name out"=w45:refnum<visa-resource-name>)  [unwired: 3 in, 2 out]
  n106 = control-ref of="Overflow?"() -> (w36:refnum<vi>)
  n107 = control-ref of="Complete?"() -> (w35:refnum<vi>)
  n108 = control-ref of="Stop"() -> (w30:refnum<vi>)
  n109 = call <instrlib>:"Display Measure Function.vi"("Function (Current)"=w39, "error in (no error)"=w46, "Channel (Channel A)"=w40, "VISA resource name"=w45) -> ("error out"=w42:errorcluster, "VISA resource name out"=w38:refnum<visa-resource-name>)  [unwired: 4 in, 2 out]
  n110 = Build Array(w36, w35, w30) -> (w34:refnum<vi>[])
  n111 = case shown="True" "Auto Enable Output" {
    tunnel: [w339 w349] -> w9
    tunnel: [w340 w348] -> w10
    tunnel: w42 -> [w339 w344]
    tunnel: w41 -> [_ w343]
    tunnel: w40 -> [_ w342]
    tunnel: w38 -> [w340 w341]
    frame False {
    }
    frame True {
      w345 = TRUE ("Output (Off)")
      n112 = call <instrlib>:"Source Output Enable.vi"("Output (Off)"=w345, "error in (no error)"=w344, "Channel (Channel A)"=w342, "VISA resource name"=w341) -> ("error out"=w347:errorcluster, "VISA resource name out"=w346:refnum<visa-resource-name>)  [unwired: 4 in, 2 out]
      n113 = call <instrlib>:"Source Output Enable.vi"("Output (Off)"=w345, "error in (no error)"=w347, "Channel (Channel A)"=w343, "VISA resource name"=w346) -> ("error out"=w349:errorcluster, "VISA resource name out"=w348:refnum<visa-resource-name>)  [unwired: 4 in, 2 out]
    }
  }
  n114 = for {
    tunnel: w34 -> [w351] mode=indexing
    tunnel: [w350] -> w31
    # "Init GUI"
    n115 = invoke class="Bool (strict)" method="Reinit To Default"(reference=w351) -> (error out=w350:errorcluster)  [unwired: 2 in, 2 out]
  }
  n116 = call <userlib>:"Wait (ms)__ogtk.vi"("error in (no error)"=w9, "milliseconds to wait"=u32 1000) -> ("error out"=w8:errorcluster)  [unwired: 8 in, 1 out]
  n117 = call <instrlib>:"Initiate Sweep.vi"("error in"=w8, "Channel (Channel A)"=w40, "VISA resource name"=w10) -> ("error out"=w70:errorcluster, "VISA resource name out"=w71:refnum<visa-resource-name>)  [unwired: 5 in, 2 out]
  n118 = Obtain Queue(max queue size (-1, unlimited)=1024, name (unnamed)="data_q", element data type=w19, error in (no error)=w42) -> (queue out=w57:refnum<queue>, error out=w32:errorcluster)  [unwired: 1 in, 1 out]
  n119 = Format Into String(format string="%s, %s, %s", "i_ds" ("Buffer Name(s)"), "i_ds.timestamps" ("Buffer Name(s)"), "v_ds" ("Buffer Name(s)")) -> (resulting string=w74:string)  [unwired: 2 in, 1 out]
  n120 = call <instrlib>:"Initiate Sweep.vi"("error in"=w70, "Channel (Channel A)"=w41, "VISA resource name"=w71) -> ("error out"=w73:errorcluster, "VISA resource name out"=w72:refnum<visa-resource-name>)  [unwired: 5 in, 2 out]
  n121 = Merge Errors(w32, w31) -> (w33:errorcluster)
  n122 = while {
    tunnel: w57 -> [w363]
    tunnel: "I_ds Log Filename" -> [w359]
    tunnel: w33 -> [w362]
    tunnel: [w358] -> w29
    shift-right: [w352] -> w15
    shift-left: w19 -> [w353]
    stop <- w356 stop-if-true
    # "Plot and save I_ds and v_ds"
    n123 = Dequeue Element(queue=w363, timeout in ms (-1)=500, error in (no error)=w362) -> (queue out=w358:refnum<queue>, element=w360:sgl[], timed out?=w361:bool, error out=w355:errorcluster)
    n124 = case shown="False" w361 {
      tunnel: w360 -> [w366 _]
      tunnel: w359 -> [w375 _]
      tunnel: [FALSE ("Operation Complete") w388] -> w354
      tunnel: w353 -> [w367 w387]
      tunnel: [w365 w387] -> w352
      frame False {
        n125 = Decimate 1D Array(w366) -> (w372:sgl[], w371:sgl[], w370:sgl[])
        n126 = for {
          tunnel: [w384] -> w374
          tunnel: [w379] -> w369 mode=indexing
          tunnel: w372 -> [w378] mode=indexing
          tunnel: w371 -> [w377] mode=indexing
          tunnel: w370 -> [w382] mode=indexing
          n127 = To Time Stamp(1:w377) -> (0:w383:timestamp)
          n128 = Build Array(w378) -> (w381:sgl[])
          n129 = Build Array(w382) -> (w380:sgl[])
          n130 = Build Array(w377, w378, w382) -> (w379:sgl[])
          "Data" <- w379
          n131 = Bundle By Name("Y"=w381, "t0"=w383) -> (w386:waveform(sgl))  [unwired: 1 in]
          n132 = Bundle By Name("Y"=w380, "t0"=w383) -> (w385:waveform(sgl))  [unwired: 1 in]
          n133 = Merge Signals(w386, w385) -> (w384:dynamicdata)
        }
        "Result Chart" <- w374
        n134 = Build Array (concatenate)(w367, w366) -> (w365:sgl[])
        n135 = call "Convert to Dynamic Data3"("2D Array"=w369) -> ("Dynamic Data Type"=w373:dynamicdata)  [unwired: 3 in]
        n136 = call "Write To Measurement File"("Signals"=w373, "Filename"=w375) -> ("Filename Out"=→"I_ds Log Filename Out":path)  [unwired: 15 in, 2 out]
      }
      frame True {
        # "Timeout and OPC = no more data, quit elegantly"
        n137 = local read "Complete?"() -> (w388:bool)
      }
    }
    n138 = local read "Stop"() -> (w357:bool)
    n139 = Compound Arithmetic op=OR(w354, w357, w355) -> (w356:bool)
  }
  n140 = while {
    tunnel: w72 -> [w397]
    tunnel: w73 -> [w396]
    shift-right: [w391] -> _
    shift-left: u32 1 ("Start Index (1)") -> [w390]
    tunnel: w74 -> [w413]
    tunnel: "tostring(i_ds.next), tostring(v_ds.next)" ("format string") -> [w411]
    tunnel: w57 -> [w395]
    tunnel: [w410] -> w61
    tunnel: [w394] -> w60
    tunnel: [w398] -> w53
    stop <- w399 stop-if-true
    # "Fetch buffer data and parse dataframes"
    n141 = Wait (ms)(milliseconds to wait=u32 100) -> ()  [unwired: 1 out]
    n142 = VISA Write(VISA resource name=w397, write buffer="*OPC", error in (no error)=w396) -> (VISA resource name out=w409:refnum<visa-resource-name>, error out=w408:errorcluster)  [unwired: 1 out]
    n143 = call <instrlib>:"ESR.vi"("error in (no error)"=w408, "VISA resource name"=w409) -> ("error out"=w403:errorcluster, "ESR"=w407:u8, "VISA resource name out"=w402:refnum<visa-resource-name>)  [unwired: 5 in, 2 out]
    n144 = And(x=w407, y=u8 1) -> (x .and. y?=w406:u8)
    n145 = Not Equal To 0?(x=w406) -> (x != 0?=w398:bool)
    "Complete?" <- w398
    n146 = call <instrlib>:"Print.vi"("Byte Count (1024)"=u32 256, "error in (no error)"=w403, "Input"=w411, "VISA resource name"=w402) -> ("error out"=w420:errorcluster, "Output"=w422:string, "VISA resource name out"=w417:refnum<visa-resource-name>)  [unwired: 3 in, 2 out]
    n147 = Scan From String(format string="%d %d", input string=w422, error in=w420) -> (error out=w416:errorcluster, output 1=w419:i32, output 2=w418:i32)  [unwired: 3 in, 2 out]
    n148 = Max & Min(x=w419, y=w418) -> (min(x,y)=w391:i32)  [unwired: 1 out]
    n149 = Decrement(x=w391) -> (x-1=w401:i32)
    n150 = Greater Or Equal?(x=w391, y=w390) -> (x >= y?=w415:bool)
    n151 = Equal?(x=w391, y=w390) -> (x = y?=w389:bool)
    n152 = case shown="False" w415 {
      tunnel: w413 -> [w429 w456]
      tunnel: w417 -> [w432 w455]
      tunnel: w416 -> [w433 w454]
      tunnel: w401 -> [w439 w453]
      tunnel: w390 -> [w446 w452]
      tunnel: u32 4096 ("Byte Count (1024)") -> [w445 w451]
      tunnel: [w435 w450] -> w393
      tunnel: [w428 w448] -> w394
      tunnel: [w427 w449] -> w410
      tunnel: w389 -> [_ w447]
      frame False {
        n153 = VISA Write(VISA resource name=w432, write buffer="i_ds.clearcache()\nv_ds.clearcache()" ("format string"), error in (no error)=w433) -> (VISA resource name out=w431:refnum<visa-resource-name>, error out=w430:errorcluster)  [unwired: 1 out]
        n154 = local read "Buffer size"() -> (w444:u32)
        n155 = call <instrlib>:"Print Buffer.vi"("VISA resource name"=w431, "Start Index (1)"=w446, "End Index (1)"=w444, "Buffer Name(s)"=w429, "error in (no error)"=w430, "Byte Count (1024)"=w445) -> ("VISA resource name out"=w442:refnum<visa-resource-name>, "Buffer Data"=w443:string, "error out"=w441:errorcluster)  [unwired: 5 in, 2 out]
        n156 = call <instrlib>:"Real 32 Converter.vi"("Data In"=w443) -> ("Data Array Out"=w437:sgl[])  [unwired: 10 in]
        n157 = call <instrlib>:"Print Buffer.vi"("VISA resource name"=w442, "Start Index (1)"=u32 1, "End Index (1)"=w439, "Buffer Name(s)"=w429, "error in (no error)"=w441) -> ("VISA resource name out"=w427:refnum<visa-resource-name>, "Buffer Data"=w438:string, "error out"=w428:errorcluster)  [unwired: 6 in, 2 out]
        n158 = call <instrlib>:"Real 32 Converter.vi"("Data In"=w438) -> ("Data Array Out"=w436:sgl[])  [unwired: 10 in]
        n159 = Build Array (concatenate)(w437, w436) -> (w435:sgl[])
      }
      frame True {
        n160 = case shown="True" w447 {
          tunnel: w456 -> [w466 _]
          tunnel: w455 -> [w465 w469]
          tunnel: w454 -> [w464 w468]
          tunnel: w453 -> [w463 _]
          tunnel: w452 -> [w462 _]
          tunnel: w451 -> [w461 _]
          tunnel: [w459 sgl[] [] ("Data Array Out")] -> w450
          tunnel: [w458 w469] -> w449
          tunnel: [w457 w468] -> w448
          frame False {
            n161 = call <instrlib>:"Print Buffer.vi"("VISA resource name"=w465, "Start Index (1)"=w462, "End Index (1)"=w463, "Buffer Name(s)"=w466, "error in (no error)"=w464, "Byte Count (1024)"=w461) -> ("VISA resource name out"=w458:refnum<visa-resource-name>, "Buffer Data"=w460:string, "error out"=w457:errorcluster)  [unwired: 5 in, 2 out]
            n162 = call <instrlib>:"Real 32 Converter.vi"("Data In"=w460) -> ("Data Array Out"=w459:sgl[])  [unwired: 10 in]
          }
          frame True {
          }
        }
      }
    }
    n163 = Empty Array?(array=w393) -> (empty?=w392:bool)
    n164 = case shown="False" w392 {
      tunnel: w395 -> [w425 _]
      tunnel: w393 -> [w424 _]
      frame False {
        n165 = Lossy Enqueue Element(queue=w425, element=w424) -> (overflow?=→"Overflow?":bool)  [unwired: 1 in, 3 out]
      }
      frame True {
      }
    }
    n166 = Or(x=w398, y="Stop") -> (x .or. y?=w399:bool)
  }
  n167 = Release Queue(queue=w29) -> (error out=w26:errorcluster)  [unwired: 2 in, 2 out]
  n168 = Decimate 1D Array(w15) -> (w18:sgl[], w17:sgl[], w16:sgl[])
  n169 = for {
    tunnel: w18 -> [w475] mode=indexing
    tunnel: w17 -> [w471] mode=indexing
    tunnel: w16 -> [w474] mode=indexing
    n170 = To Time Stamp(1:w471) -> (0:w476:timestamp)
    n171 = Build Array(w475) -> (w473:sgl[])
    n172 = Build Array(w474) -> (w472:sgl[])
    n173 = Bundle By Name("Y"=w473, "t0"=w476) -> (w478:waveform(sgl))  [unwired: 1 in]
    n174 = Bundle By Name("Y"=w472, "t0"=w476) -> (w477:waveform(sgl))  [unwired: 1 in]
    n175 = Merge Signals(w478, w477) -> (w470:dynamicdata)
    n176 = local write "Result Chart"(w470) -> ()
  }
  n177 = case shown="False" w53 {
    tunnel: w61 -> [w486 w488]
    tunnel: w60 -> [w485 w487]
    tunnel: [w480 w488] -> w59
    tunnel: [w479 w487] -> w58
    frame False {
      w481 = u16 1 items=["Channel A", "Channel B"] ("Channel (Channel A)")
      w482 = u16 0 items=["Channel A", "Channel B"] ("Channel (Channel A)")
      # "Abort Operation"
      n178 = call <instrlib>:"Abort SMU Op.vi"("error in"=w485, "Channel (Channel A)"=w482, "VISA resource name"=w486) -> ("error out"=w483:errorcluster, "VISA resource name out"=w484:refnum<visa-resource-name>)  [unwired: 5 in, 2 out]
      n179 = call <instrlib>:"Abort SMU Op.vi"("error in"=w483, "Channel (Channel A)"=w481, "VISA resource name"=w484) -> ("error out"=w479:errorcluster, "VISA resource name out"=w480:refnum<visa-resource-name>)  [unwired: 5 in, 2 out]
    }
    frame True {
      # "Operation Completed"
    }
  }
  n180 = local read "Auto Enable Output"() -> (w11:bool)
  n181 = case shown="False" w11 {
    tunnel: w59 -> [w490 w494]
    tunnel: w58 -> [w489 w493]
    tunnel: [w489 w492] -> w55
    tunnel: [w490 w491] -> w54
    frame False {
    }
    frame True {
      w499 = FALSE ("Output (Off)")
      n182 = local read "Drain Source Channel"() -> (w496:T1)
      n183 = local read "Pulse Channel"() -> (w495:T1)
      n184 = call <instrlib>:"Source Output Enable.vi"("Output (Off)"=w499, "error in (no error)"=w493, "Channel (Channel A)"=w496, "VISA resource name"=w494) -> ("error out"=w497:errorcluster, "VISA resource name out"=w498:refnum<visa-resource-name>)  [unwired: 4 in, 2 out]
      n185 = call <instrlib>:"Source Output Enable.vi"("Output (Off)"=w499, "error in (no error)"=w497, "Channel (Channel A)"=w495, "VISA resource name"=w498) -> ("error out"=w492:errorcluster, "VISA resource name out"=w491:refnum<visa-resource-name>)  [unwired: 4 in, 2 out]
    }
  }
  n186 = case shown="True" w53 {
    tunnel: w55 -> [w500 w519]
    tunnel: w54 -> [w501 w518]
    tunnel: [w500 w507] -> w52
    tunnel: [w501 w513] -> w51
    frame False {
      # "Operation Aborted, do nothing"
    }
    frame True {
      # "Plot and save Pulsed IV (single point)"
      n187 = local read "LT Pulse Number"() -> (w515:u32)
      n188 = call <instrlib>:"Print Buffer.vi"("VISA resource name"=w518, "End Index (1)"=w515, "Buffer Name(s)"="pulse_iv_table.v, pulse_iv_table.i" ("Buffer Name (buf)"), "error in (no error)"=w519, "Byte Count (1024)"=u32 4096) -> ("VISA resource name out"=w513:refnum<visa-resource-name>, "Buffer Data"=w514:string, "error out"=w508:errorcluster)  [unwired: 6 in, 2 out]
      n189 = call <instrlib>:"Real 32 Converter.vi"("Data In"=w514) -> ("Data Array Out"=w512:sgl[])  [unwired: 10 in]
      n190 = Decimate 1D Array(w512) -> (w511:sgl[], w510:sgl[])
      n191 = call "Convert to Dynamic Data2"("Array"=w510) -> ("Dynamic Data Type"=w505:dynamicdata)  [unwired: 3 in]
      n192 = call "Convert to Dynamic Data"("Array"=w511) -> ("Dynamic Data Type"=w506:dynamicdata)  [unwired: 3 in]
      n193 = Merge Signals(w506, w505) -> (w502:dynamicdata)
      n194 = call "Build XY Graph"("error in (no error)"=w508, "Y Input"=w505, "X Input"=w506) -> ("error out"=w507:errorcluster, "XY Graph"=→"Pulse IV":cluster{"X":dbl[], "Y":dbl[]}[])  [unwired: 7 in]
      n195 = call "Write To Measurement File2"("Signals"=w502, "Filename"="Pulsed IV Filename") -> ("Filename Out"=→"Pulsed IV Filename Out":path)  [unwired: 15 in, 2 out]
    }
  }
  n196 = call <instrlib>:"Close.vi"("error in (no error)"=w52, "VISA resource name"=w51) -> ("error out"=w28:errorcluster)  [unwired: 9 in]
  n197 = Merge Errors(w28, w26) -> (→"error out":errorcluster)
